vi "[ce] Open Probe VI Reference.vi"(8 "error in":errorcluster, 10 "VI instance name":string, 11 "master VI name":string) -> (0 "error out":errorcluster, 3 "vi refnum":refnum<vi>, 4 "new window?":bool)   [LabVIEW 2021]
doc: "::: CalcExpress Toolkit :::\nCopyright (c) 2000-2026 Konstantin Shifershteyn. All rights reserved."
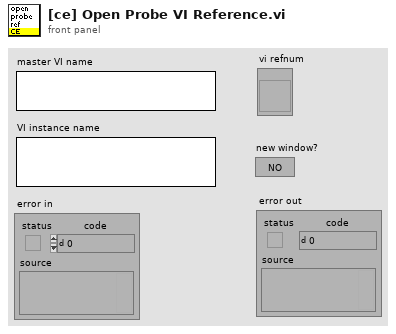
[diagram p1: front panel]
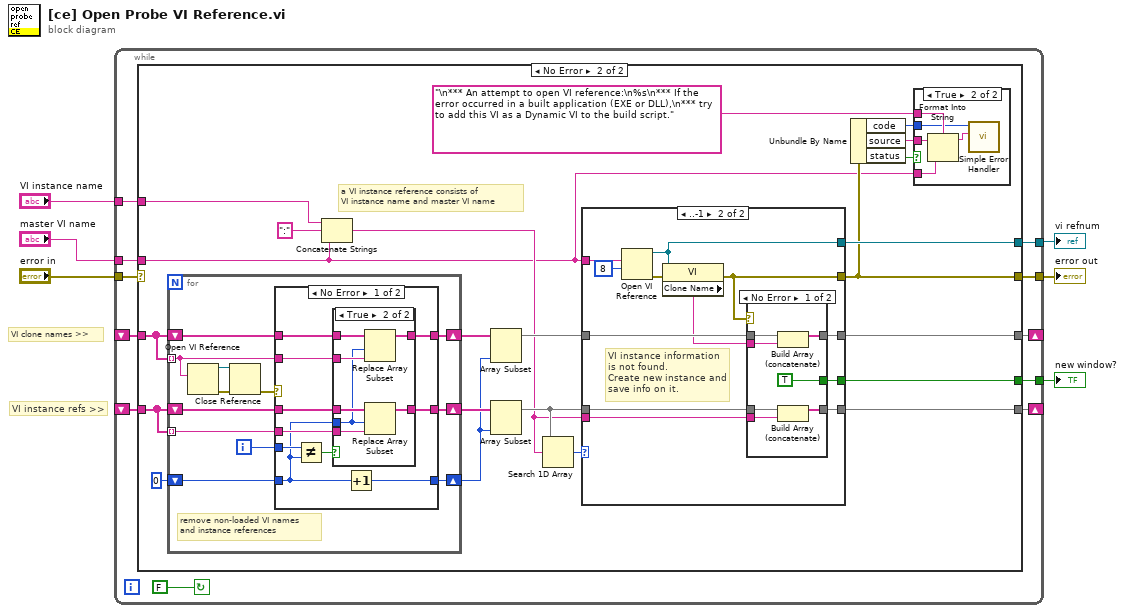
[diagram p0: block diagram]
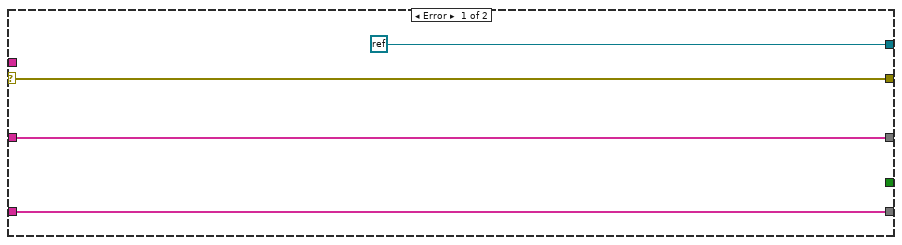
[diagram p2: hidden frame]
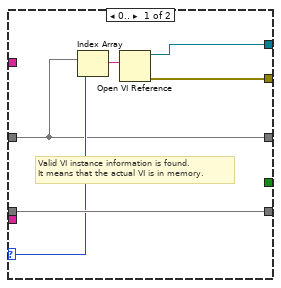
[diagram p4: hidden frame]
diagram:
  # "VI instance refs >>"
  # "VI clone names >>"
  n1 = while {
    tunnel: [w12] -> w5
    tunnel: [w13] -> w4
    tunnel: "error in" -> [w10]
    shift-left: _ -> [w17]
    shift-right: [w14] -> _
    shift-left: _ -> [w16]
    shift-right: [w15] -> _
    tunnel: [w9] -> w3
    tunnel: "VI instance name" -> [w8]
    tunnel: "master VI name" -> [w7]
    stop <- FALSE continue-if-true
    n2 = case shown="No Error" w10 {
      selector: w10 -> [w18 _]
      tunnel: w17 -> [w20 w32]
      tunnel: w16 -> [w21 w31]
      tunnel: [w21 w38] -> w15
      tunnel: [w20 w36] -> w14
      tunnel: [w18 w25] -> w13
      tunnel: [refnum<k0> refnum ("Not a Refnum Constant") w33] -> w12
      tunnel: [_ w24] -> w9
      tunnel: w8 -> [_ w23]
      tunnel: w7 -> [_ w22]
      frame Error {
      }
      frame No Error {
        # "a VI instance reference consists of\nVI instance name and master VI name"
        n3 = for {
          shift-right: [w85] -> w41
          shift-left: w32 -> [w84]
          shift-right: [w77] -> w40
          shift-left: 0 -> [w78]
          shift-right: [w83] -> w42
          shift-left: w31 -> [w82]
          tunnel: w32 -> [w81] mode=indexing
          tunnel: w31 -> [w80] mode=indexing
          i -> [w76]
          # "remove non-loaded VI names\nand instance references"
          n4 = Open VI Reference(vi path=w80) -> (vi reference=w87:refnum<vi>, error out=w86:errorcluster)  [unwired: 5 in]
          n5 = Close Reference(reference=w87, error in (no error)=w86) -> (error out=w79:errorcluster)
          n6 = case shown="No Error" w79 {
            tunnel: w84 -> [w97 w109]
            tunnel: [w96 w109] -> w85
            tunnel: w81 -> [w95 _]
            tunnel: w82 -> [w94 w108]
            tunnel: [w93 w108] -> w83
            tunnel: w80 -> [w92 _]
            tunnel: w78 -> [w88 w107]
            tunnel: [w91 w107] -> w77
            tunnel: w76 -> [w90 _]
            frame No Error {
              n7 = Not Equal?(x=w90, y=w88) -> (x != y?=w89:bool)
              n8 = case shown="True" w89 {
                tunnel: w97 -> [w98 w106]
                tunnel: [w98 w105] -> w96
                tunnel: w95 -> [_ w104]
                tunnel: w94 -> [w99 w103]
                tunnel: [w99 w102] -> w93
                tunnel: w92 -> [_ w101]
                tunnel: w88 -> [_ w100]
                frame False {
                }
                frame True {
                  n9 = Replace Array Subset(array=w103, new element=w101, index=w100) -> (w102:string[])
                  n10 = Replace Array Subset(array=w106, new element=w104, index=w100) -> (w105:string[])
                }
              }
              n11 = Increment(x=w88) -> (x+1=w91:i32)
            }
            frame Error {
            }
          }
        }
        n12 = Concatenate Strings(w23, ":", w22) -> (w34:string)
        n13 = Array Subset(array=w42, length=w40) -> (w37:string[])  [unwired: 1 in]
        n14 = Array Subset(array=w41, length=w40) -> (w35:string[])  [unwired: 1 in]
        n15 = Search 1D Array(1D array=w35, element=w34) -> (index of element=w30:i32)  [unwired: 1 in]
        n16 = case shown="..-1" w30 {
          selector: w30 -> [w53 _]
          tunnel: w22 -> [_ w65]
          tunnel: [w52 w64] -> w38
          tunnel: w37 -> [w52 w63]
          tunnel: w35 -> [w54 w61]
          tunnel: [w54 w62] -> w36
          tunnel: w34 -> [_ w60]
          tunnel: [w50 w55] -> w25
          tunnel: [w49 w58] -> w33
          tunnel: [_ w56] -> w24
          frame 0.. {
            # "Valid VI instance information is found.\nIt means that the actual VI is in memory."
            n17 = Index Array(array=w52, index=w53) -> (element=w51:string)
            n18 = Open VI Reference(vi path=w51) -> (vi reference=w49:refnum<vi>, error out=w50:errorcluster)  [unwired: 5 in]
          }
          frame ..-1 {
            # "VI instance information\nis not found.\nCreate new instance and\nsave info on it."
            n19 = Open VI Reference(vi path=w65, options=8) -> (vi reference=w58:refnum<vi>, error out=w66:errorcluster)  [unwired: 4 in]
            n20 = property on="vi name" class="VI"(reference=w58, error in=w66) -> (error out=w55:errorcluster, "Clone Name"=w59:string)  [unwired: 1 out]
            n21 = case shown="No Error" w55 {
              tunnel: [w73 w75] -> w64
              tunnel: w63 -> [w72 w75]
              tunnel: w59 -> [w71 _]
              tunnel: [w70 w74] -> w62
              tunnel: w61 -> [w69 w74]
              tunnel: w60 -> [w68 _]
              tunnel: [TRUE _] -> w56
              frame No Error {
                n22 = Build Array (concatenate)(w72, w71) -> (w73:string[])
                n23 = Build Array (concatenate)(w69, w68) -> (w70:string[])
              }
              frame Error {
              }
            }
          }
        }
        n24 = Unbundle By Name(w25) -> ("code"=w28:i32, "source"=w29:string, "status"=w27:bool)
        n25 = case shown="True" w27 {
          tunnel: w29 -> [_ w48]
          tunnel: w22 -> [_ w47]
          tunnel: "\n*** An attempt to open VI reference:\n%s\n*** If the error occurred in a built application (EXE or DLL),\n*** try to add this VI as a Dynamic VI to the build script." -> [_ w46]
          tunnel: w28 -> [_ w45]
          frame False {
          }
          frame True {
            n26 = Format Into String(format string=w46, initial string=w48, w47) -> (resulting string=w44:string)  [unwired: 1 in, 1 out]
            n27 = call <vilib>:"Simple Error Handler.vi"("error code (no error:0)"=w45, "error source (\" \")"=w44) -> ()  [unwired: 3 in, 5 out]
          }
        }
      }
    }
  }
  "error out" <- w4
  "vi refnum" <- w5
  "new window?" <- w3
